vi "TestUI.vi"() -> ()   [LabVIEW 2021]
uses:
  Dependencies/Channel.lvlibp
  <vilib>/ActorFramework/Actor/Actor.lvclass
  Dependencies/Channel.lvlibp/Channel/ChannelManagerUI/ChannelManagerUI.lvclass
  C:/Users/averna/Documents/LV Gym DEMO/Factory Pattern/Channels/Dependencies/Channel.lvlibp/Channel/ChannelsManager/ChannelsManager/ChannelsManager.lvclass
  C:/Users/averna/Documents/LV Gym DEMO/Factory Pattern/Channels/Dependencies/Channel.lvlibp/1abvi3w/vi.lib/ActorFramework/Actor/Actor.lvclass
  C:/Users/averna/Documents/LV Gym DEMO/Factory Pattern/Channels/Dependencies/Channel.lvlibp/Channel/ChannelManagerUI/ChannelManagerUI.lvclass
panel:
  in  "Config File":path=path "C:/Users/averna/Documents/LV Gym DEMO/Factory Pattern/Channels/Files/Test.ini"
  in  "Plugins Folder":path=path "C:/Users/averna/Documents/LV Gym DEMO/Factory Pattern"
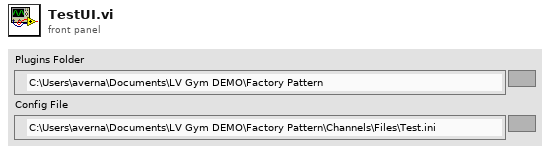
[diagram p1: front panel]
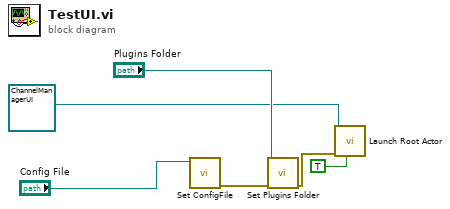
[diagram p0: block diagram]
diagram:
  n1 = call "Set ConfigFile.vi"("Plugins Folder"="Config File") -> ("error out"=w6:errorcluster)  [unwired: 10 in]
  n2 = call "Set Plugins Folder.vi"("error in (no error)"=w6, "Config File"="Plugins Folder") -> ("error out"=w2:errorcluster)  [unwired: 9 in]
  n3 = call <vilib>:"Launch Root Actor.vi"("Open Actor Core front panel? (F)"=TRUE, "error in (no error)"=w2, "Actor"=refnum<class "ChannelManagerUI.lvclass"> refnum ("Channel.lvlibp:ChannelManagerUI.lvlib:ChannelManagerUI")) -> ()  [unwired: 7 in, 2 out]
